vi "AssertNotEqual_Tests.vi"(11 "error in":errorcluster) -> (15 "error out":errorcluster)   [LabVIEW 2016, in "DronaTest.lvlib"]
uses:
  DronaTest.lvlib
  APIs/Assert/AssertControlValue/NotEqual.vi
  <vilib>/addons/_JKI Toolkits/Caraya/classes/Assert/Assert Not Equal Value_Variant.vi
  <vilib>/addons/_JKI Toolkits/Caraya/classes/Assert/Assert Error.vi
  <vilib>/addons/_JKI Toolkits/Caraya/classes/Test/Test.lvclass
  Drona.lvlib
  <vilib>/addons/_JKI Toolkits/Caraya/classes/Assert/Assert.lvclass
  APIs/Assert/AssertControlValue/AssertControlValue.lvlib
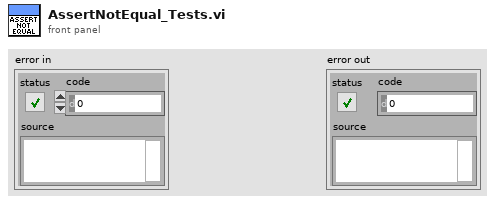
[diagram p1: front panel]
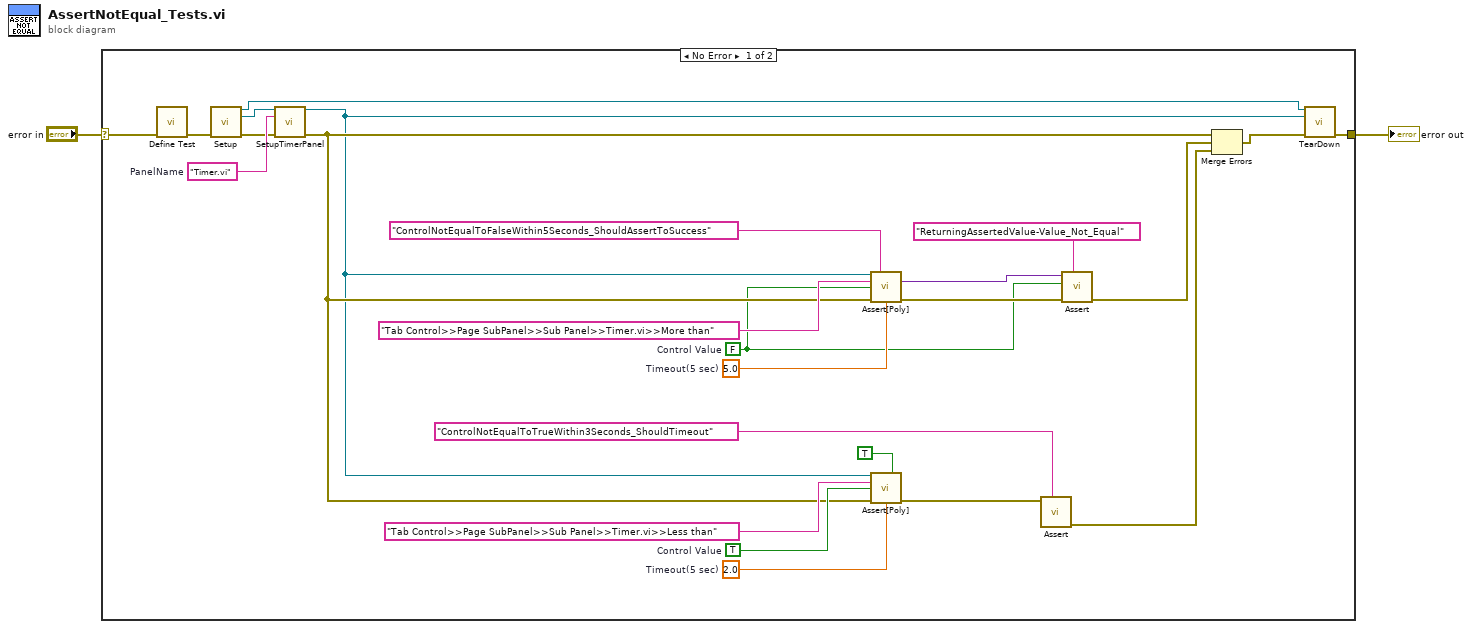
[diagram p0: block diagram]
diagram:
  n1 = case shown="No Error" "error in" {
    selector: "error in" -> [w27 w28]
    tunnel: [w9 w28] -> w1
    frame No Error {
      w16 = "Timer.vi"  # PanelName
      w17 = TRUE  # Control Value
      w22 = 2.0  # Timeout(5 sec)
      w21 = 5.0  # Timeout(5 sec)
      w4 = FALSE  # Control Value
      n2 = call <vilib>:"Define Test.vi"("error in (no error)"=w27) -> ("error out"=w15:errorcluster)  [unwired: 9 in, 1 out]
      n3 = call "Setup.vi"("error in (no error)"=w15) -> ("Application Ref"=w12:refnum<vi>, "VI out"=w13:refnum<vi>, "error out"=w14:errorcluster)  [unwired: 12 in]
      n4 = call "SetupTimerPanel.vi"("VI in"=w13, "Item Name"=w16, "error in (no error)"=w14) -> ("VI out"=w8:refnum<vi>, "error out"=w11:errorcluster)  [unwired: 11 in]
      n5 = call-poly "Assert[Poly].vi"("VI Reference In"=w8, "Test Label"="ControlNotEqualToFalseWithin5Seconds_ShouldAssertToSuccess" ("string"), "Control Path"="Tab Control>>Page SubPanel>>Sub Panel>>Timer.vi>>More than", "Control Value"=w4, "Error In"=w11, "Timeout(5 sec)"=w21) -> ("Asserted Value"=w5:variant, "Error Out"=w7:errorcluster)  [unwired: 7 in, 1 out]
      n6 = call-poly "Assert[Poly].vi"("VI Reference In"=w8, "Assert Only? (F)"=TRUE, "Control Path"="Tab Control>>Page SubPanel>>Sub Panel>>Timer.vi>>Less than", "Control Value"=w17, "Error In"=w11, "Timeout(5 sec)"=w22) -> ("Error Out"=w24:errorcluster)  [unwired: 7 in, 2 out]
      n7 = call-poly <vilib>:"Assert.vi"("Label"="ControlNotEqualToTrueWithin3Seconds_ShouldTimeout" ("string"), "Error?"=w24) -> ("error out"=w18:errorcluster)  [unwired: 8 in, 1 out]
      n8 = call-poly <vilib>:"Assert.vi"("Label"="ReturningAssertedValue-Value_Not_Equal", "error in (no error)"=w7, "Y"=w4, "X"=w5) -> ("error out"=w6:errorcluster)  [unwired: 6 in, 1 out]
      n9 = Merge Errors(w11, w6, w18) -> (w10:errorcluster)
      n10 = call "TearDown.vi"("Application Ref"=w12, "VI in"=w8, "error in (no error)"=w10) -> ("error out"=w9:errorcluster)  [unwired: 12 in]
    }
    frame Error {
    }
  }
  "error out" <- w1
